vi "LinearPlntInvFF_Calculate.vi"(9 "NextR":T1, 10 "R":T1, 11 "Input Linear Plant Inv FF":T2) -> (0 "Error":bool, 2 "Uff":T1, 3 "Output Linear Plant Inv FF":T2)   [LabVIEW 2019, in "Trajectory_Library.lvlib"]
doc: "Calculate the feedforward with current and future reference vectors.\n \nInputs:\n - LinearPlntInversionFF -- system data cluster\n - r -- The reference state of the current timestep (k).\n - nextR -- The reference state of the future timestep (k + dt).\n\nOutputs:\n - outLinearPlntInversionFF -- updated system data cluster\n - Uff -- The calculated feedforward.\n - error -- If TRUE, an error occured."
uses:
  Trajectory_Library.lvlib
  <vilib>/Analysis/NI_AALBase.lvlib
  <vilib>/Analysis/baseanly.llb/Real A x B.vi
  <vilib>/Analysis/NI_AALPro.lvlib
  <vilib>/Analysis/7linalg.llb/Solve Linear Equations (multiple right hand).vi
  <vilib>/Analysis/Matrix/NI_Matrix.lvlib
  <vilib>/Analysis/Matrix/Numeric/Subtract/Subtract - RM,RM.vi
  <vilib>/Analysis/Matrix/Datatypes/RealMatrix.ctl
  TypeDef/LINEAR_PLANT_INV_FF.ctl
panel:
  # "<States,1>"
  # "<Inputs,1>"
  # "<States,Inputs>"
  # "<States,States>"
  # "<States,1>"
  # "<Inputs,1>"
  # "<States,Inputs>"
  # "<States,States>"
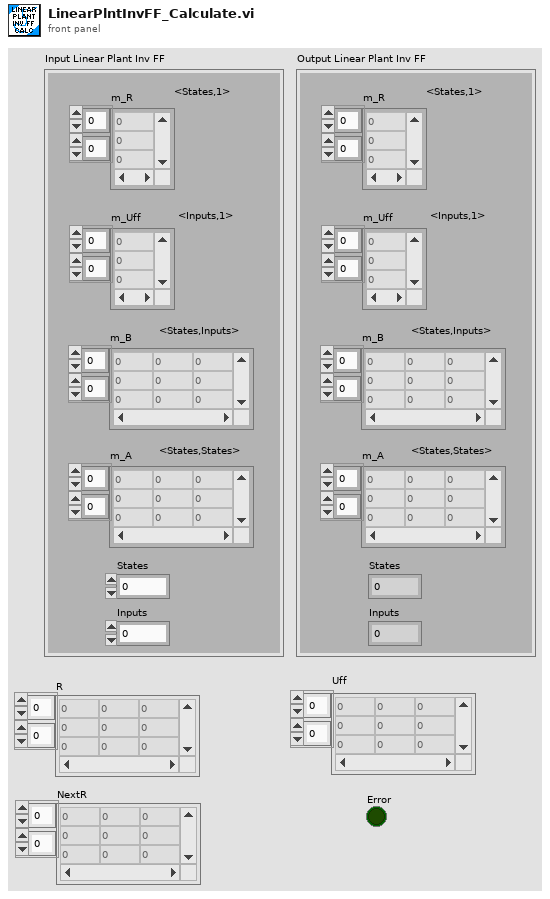
[diagram p1: front panel]
types:
  T1 = typedef "NI_Matrix.lvlib/RealMatrix.ctl" = dbl[][]
  T2 = typedef "Trajectory_Library.lvlib/LINEAR_PLANT_INV_FF.ctl" = cluster{"m_R":T1, "m_Uff":T1, "m_B":T1, "m_A":T1, "States":i32, "Inputs":i32}
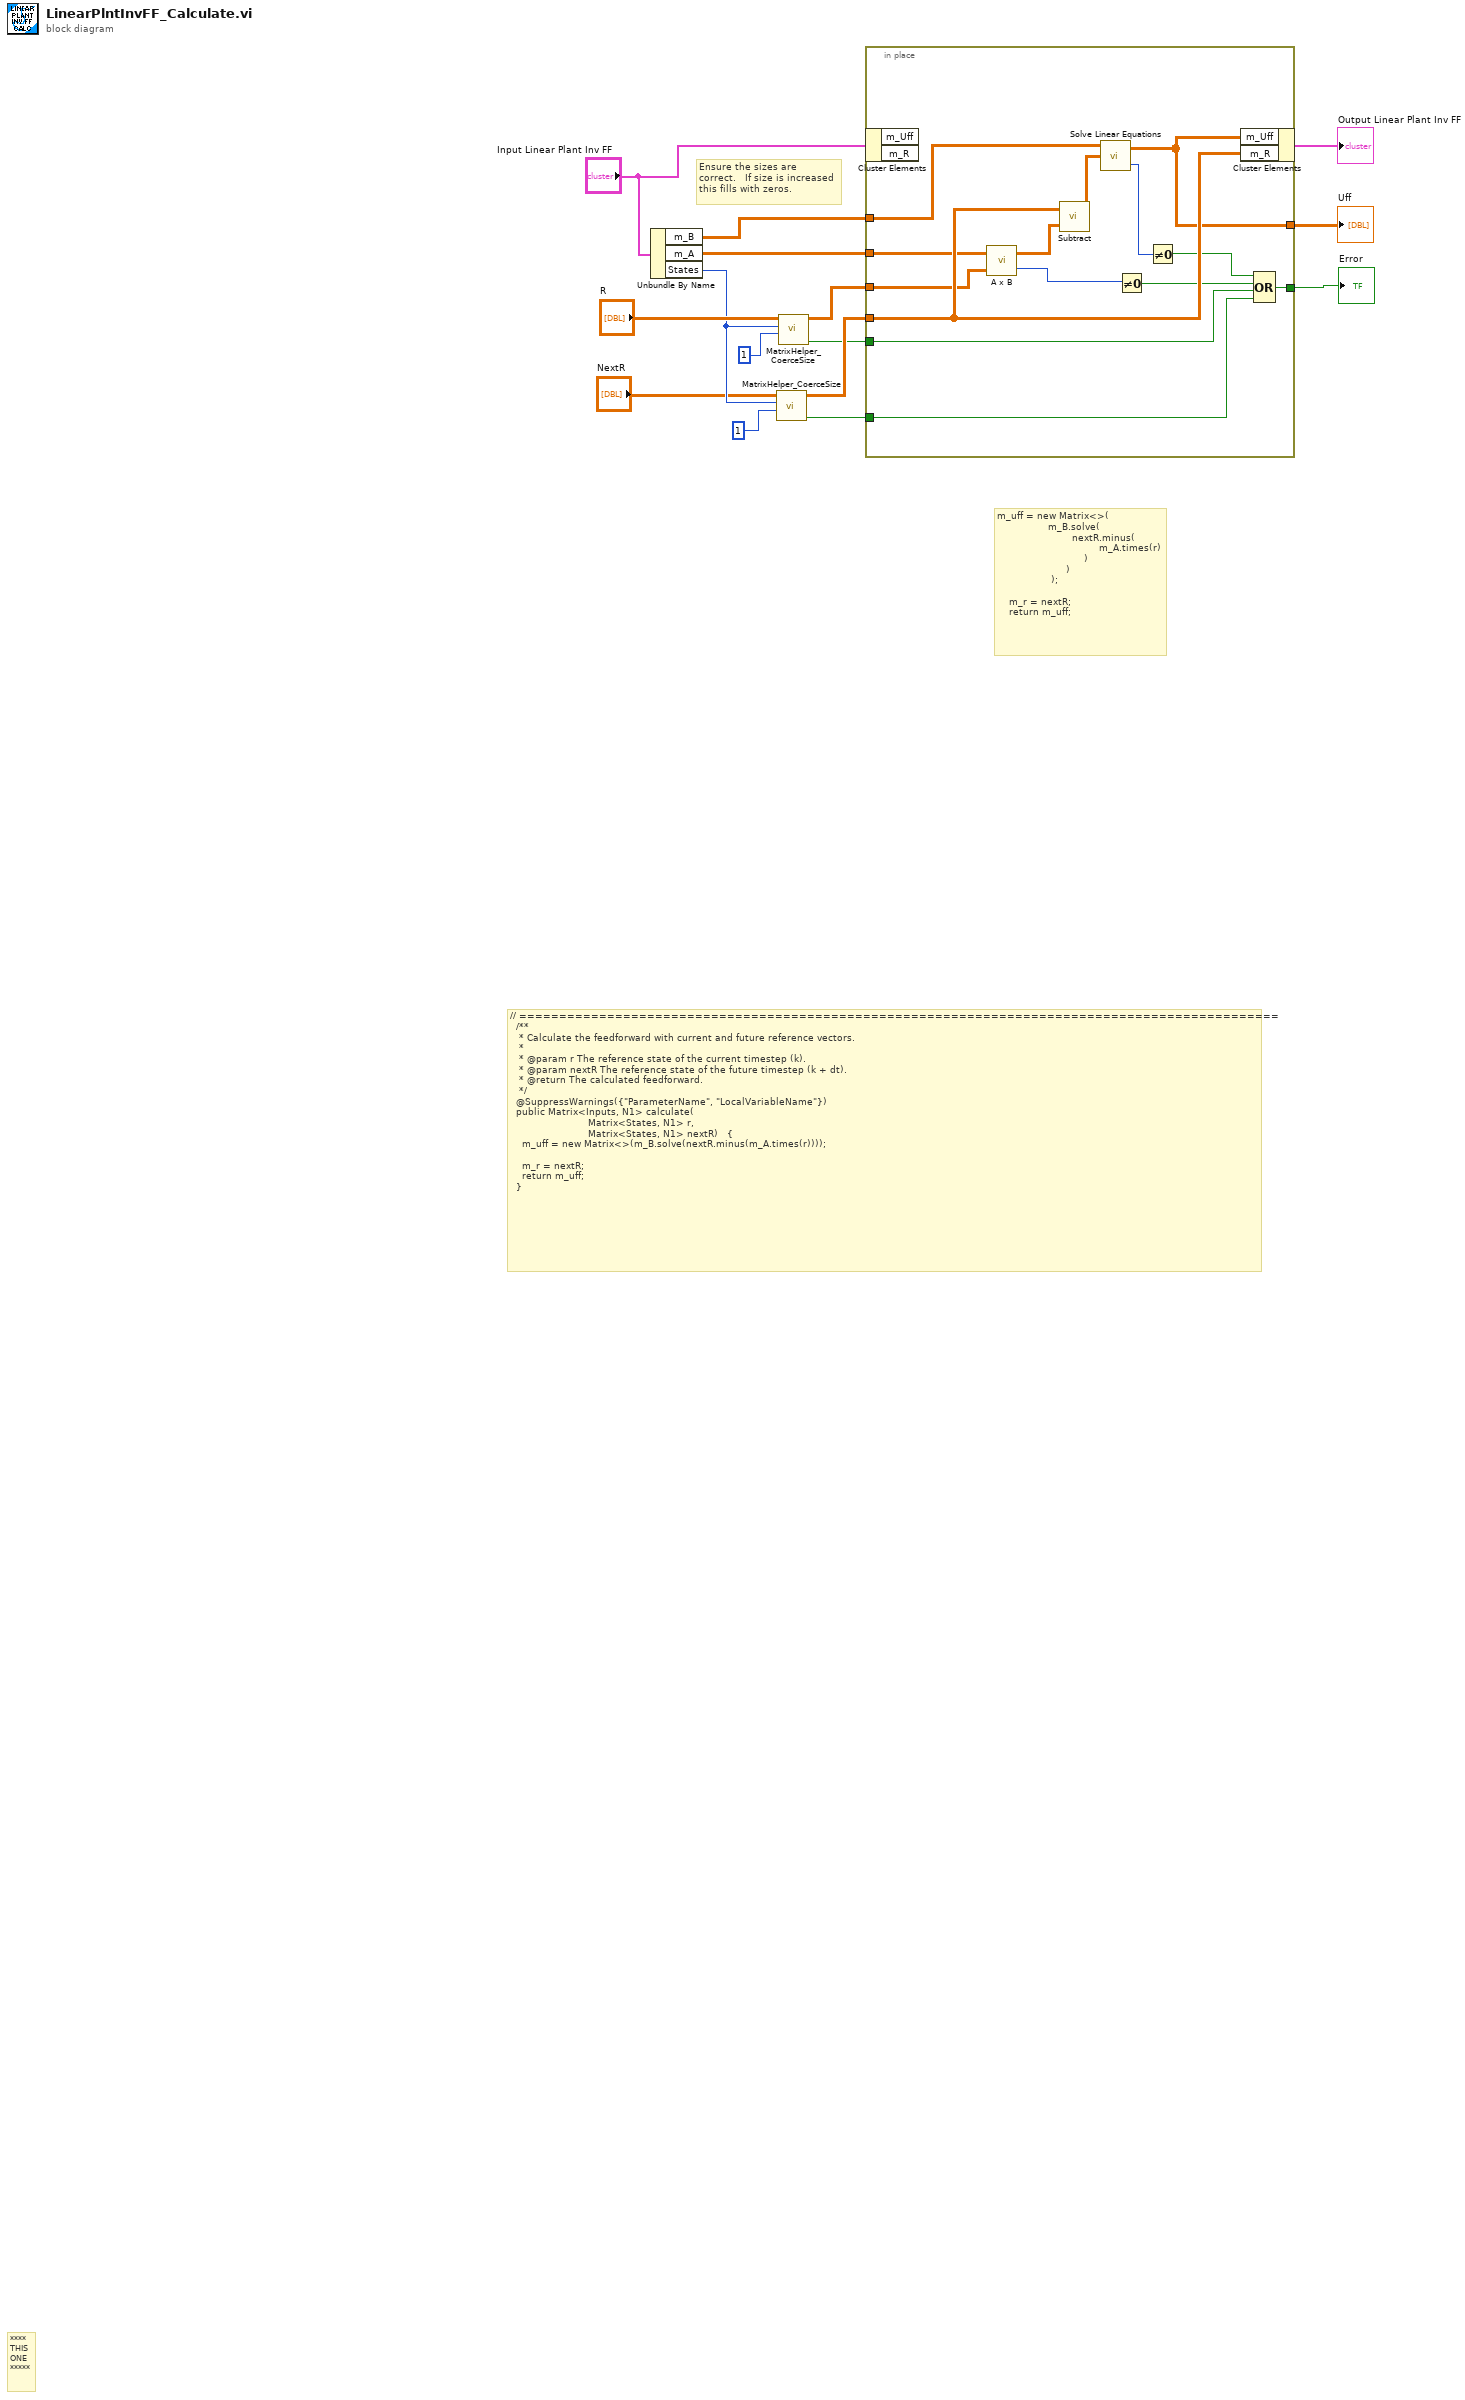
[diagram p0: block diagram]
diagram:
  # "m_uff = new Matrix<>(\n                 m_B.solve(\n                         nextR.minus(\n                                  m_A.times(r) \n                             )\n                       )\n                  );\n\n    m_r = nextR;\n    return m_uff;"
  # "// ===============================================================================================\n  /**\n   * Calculate the feedforward with current and future reference vectors.\n   *\n   * @param r The reference state of the current timestep (k).\n   * @param nextR The reference state of the future timestep (k + dt).\n   * @return The calculated feedforward.\n   */\n  @SuppressWarnings({\"ParameterName\", \"LocalVariableName\"})\n  public Matrix<Inputs, N1> calculate(\n                          Matrix<States, N1> r, \n                          Matrix<States, N1> nextR)   {\n    m_uff = new Matrix<>(m_B.solve(nextR.minus(m_A.times(r))));\n\n    m_r = nextR;\n    return m_uff;\n  }"
  # "Ensure the sizes are\ncorrect.   If size is increased \nthis fills with zeros."
  # "****\nTHIS\nONE\n*****"
  n1 = Unbundle By Name("Input Linear Plant Inv FF") -> ("m_B"=w13:T1, "m_A"=w14:T1, "States"=w6:i32)
  n2 = call "MatrixHelper_CoerceSize.vi"("Columns"=1 ("y"), "Rows"=w6, "input matrix"="NextR") -> ("Coerced"=w1:bool, "output matrix"=w3:T1)  [unwired: 7 in]
  n3 = call "MatrixHelper_CoerceSize.vi"("Columns"=1 ("y"), "Rows"=w6, "input matrix"="R") -> ("Coerced"=w2:bool, "output matrix"=w7:T1)  [unwired: 7 in]
  n4 = in-place {
    in-place-border: w3 -> [w29]
    in-place-border: w14 -> [w28]
    in-place-border: w7 -> [w27]
    in-place-border: w13 -> [w24]
    in-place-border: [w23] -> w11
    in-place-border: [w18] -> w10
    in-place-border: w2 -> [w17]
    in-place-border: w1 -> [w16]
    n5 = in-place-cluster #1("Input Linear Plant Inv FF") -> ()  [unwired: 2 out]
    n6 = call-poly <vilib>:"A x B.vi"("B"=w27, "A"=w28) -> ("error"=w22:i32, "A x B"=w26:T1)
    n7 = call-poly <vilib>:"Subtract.vi"("Real Matrix B"=w26, "Real Matrix A"=w29) -> ("A - B"=w25:T1)
    n8 = call-poly <vilib>:"Solve Linear Equations.vi"("Known Matrix"=w25, "Input Matrix"=w24) -> ("error"=w21:i32, "Solution Matrix"=w23:T1)  [unwired: 1 in]
    n9 = Not Equal To 0?(x=w22) -> (x != 0?=w19:bool)
    n10 = Not Equal To 0?(x=w21) -> (x != 0?=w20:bool)
    n11 = in-place-cluster #1("m_Uff"=w23, "m_R"=w29) -> (→"Output Linear Plant Inv FF":T2)
    n12 = Compound Arithmetic op=OR(w20, w19, w17, w16) -> (w18:bool)
  }
  "Uff" <- w11
  "Error" <- w10
